vi "Ecrire_fichier_rapport_profil_EPC3000.vi"(1 "Commentaires":string, 4 "Chemin du fichier rapport":path) -> (5 "annulé":bool, 7 "error out":errorcluster caption="sortie d'erreur")   [LabVIEW 2022 SP3]
uses:
  Enum/Enum r3.ctl
  <vilib>/Utility/miscctls.llb/LVDateTimeRec.ctl
  <vilib>/printing/EasyPrintingControls.llb/layout_options.ctl
  <vilib>/printing/EasyPrintingControls.llb/orientation.ctl
  <vilib>/printing/EasyPrintingControls.llb/panel_scaling_for_page.ctl
  <vilib>/printing/EasyPrintingControls.llb/margins.ctl
  <vilib>/printing/EasyPrintingControls.llb/margin_values.ctl
  <vilib>/printing/EasyPrintingControls.llb/measurement_system.ctl
  <vilib>/printing/EasyPrintingControls.llb/printer_options.ctl
  <vilib>/printing/EasyPrintingControls.llb/printing_method.ctl
  <vilib>/printing/EasyPrintingControls.llb/color_or_monochrome.ctl
  <vilib>/printing/EasyPrintingControls.llb/page_header_options.ctl
  <vilib>/printing/EasyPrintingControls.llb/page_headers.ctl
  <vilib>/printing/EasyPrintingControls.llb/page_header_content_options.ctl
  <vilib>/printing/EasyPrintingControls.llb/contents.ctl
  <vilib>/printing/EasyPrintingControls.llb/report_type.ctl
  <vilib>/Utility/NIReport.llb/HTML Report Image Alignment.ctl
  Variables globales/Variables glob EUROTHERM.vi
  <vilib>/printing/EasyPrinting.llb/Print VI Panel or Documentation (path).vi
  <vilib>/Utility/NIReport.llb/Append Report Text (str wrap).vi
  <vilib>/Utility/NIReport.llb/Append Image to Report (path wrap).vi
  <vilib>/Utility/NIReport.llb/NI_report.lvclass
  <vilib>/Utility/NIReport.llb/NI_ReportGenerationCore.lvlib
panel:
  in  "Annuler lecture reg":bool
  in  "imprimer":bool
  in  "Bascule":bool
  out "nb profils":i32
  in  "Commande onglets":T1(tab)
  in  "Tinit reg 1":u16(ring) caption="Tinit sur reg :" items=["centre", "arrière"]
  out "Graph 1":cluster{"Y":dbl[], "Y":dbl[]}[](graph) caption="Profil"
  out "Régulateurs 1":string[](array[string]) caption="Régulateurs"
  out "Listing - 1":string caption="Listing programmes"
  out "Graph 2":cluster{"Y":dbl[], "Y":dbl[]}[](graph) caption="Profil"
  out "Régulateurs 2":string[](array[string]) caption="Régulateurs"
  in  "Tinit reg 2":u16(ring) caption="Tinit sur reg :" items=["EPC3008"]
  out "Listing - 2":string caption="Listing programmes"
  in  "Tinit reg 3":u16(ring) caption="Tinit sur reg :"
  out "Graph 3":cluster{"Y":dbl[], "Y":dbl[]}[](graph) caption="Profil"
  out "Régulateurs 3":string[](array[string]) caption="Régulateurs"
  out "Listing - 3":string caption="Listing programmes"
  in  "Tinit reg 4":u16(ring) caption="Tinit sur reg :"
  out "Graph 4":cluster{"Y":dbl[], "Y":dbl[]}[](graph) caption="Profil"
  out "Régulateurs 4":string[](array[string]) caption="Régulateurs"
  out "Listing - 4":string caption="Listing programmes"
  in  "Tinit reg 5":u16(ring) caption="Tinit sur reg :"
  out "Graph 5":cluster{"Y":dbl[], "Y":dbl[]}[](graph) caption="Profil"
  out "Régulateurs 5":string[](array[string]) caption="Régulateurs"
  out "Listing - 5":string caption="Listing programmes"
  in  "Tinit reg 6":u16(ring) caption="Tinit sur reg :"
  out "Graph 6":cluster{"Y":dbl[], "Y":dbl[]}[](graph) caption="Profil"
  out "Régulateurs 6":string[](array[string]) caption="Régulateurs"
  out "Listing - 6":string caption="Listing programmes"
  in  "Tinit reg 7":u16(ring) caption="Tinit sur reg :"
  out "Graph 7":cluster{"Y":dbl[], "Y":dbl[]}[](graph) caption="Profil"
  out "Régulateurs 7":string[](array[string]) caption="Régulateurs"
  out "Listing - 7":string caption="Listing programmes"
  in  "Tinit reg 8":u16(ring) caption="Tinit sur reg :"
  out "Graph 8":cluster{"Y":dbl[], "Y":dbl[]}[](graph) caption="Profil"
  out "Régulateurs 8":string[](array[string]) caption="Régulateurs"
  out "Listing - 8":string caption="Listing programmes"
  in  "Tinit reg 9":u16(ring) caption="Tinit sur reg :"
  out "Graph 9":cluster{"Y":dbl[], "Y":dbl[]}[](graph) caption="Profil"
  out "Régulateurs 9":string[](array[string]) caption="Régulateurs"
  out "Listing - 9":string caption="Listing programmes"
  in  "Tinit reg 10":u16(ring) caption="Tinit sur reg :"
  out "Graph 10":cluster{"Y":dbl[], "Y":dbl[]}[](graph) caption="Profil"
  out "Régulateurs 10":string[](array[string]) caption="Régulateurs"
  out "Listing - 10":string caption="Listing programmes"
  out "fichiers images":path[](array[path])
  in  "Annuler":bool
  in  "OK":bool
  out "Listings":string[](array[string])
  out "Profils":T2(array[cluster])
  out "Chaîne":string
  # "Ce logiciel et les informations qu'il contient, sont la propriété de l’IAS et ne peuvent être diffusés sans l’autorisation de la Station d’étalonnage"
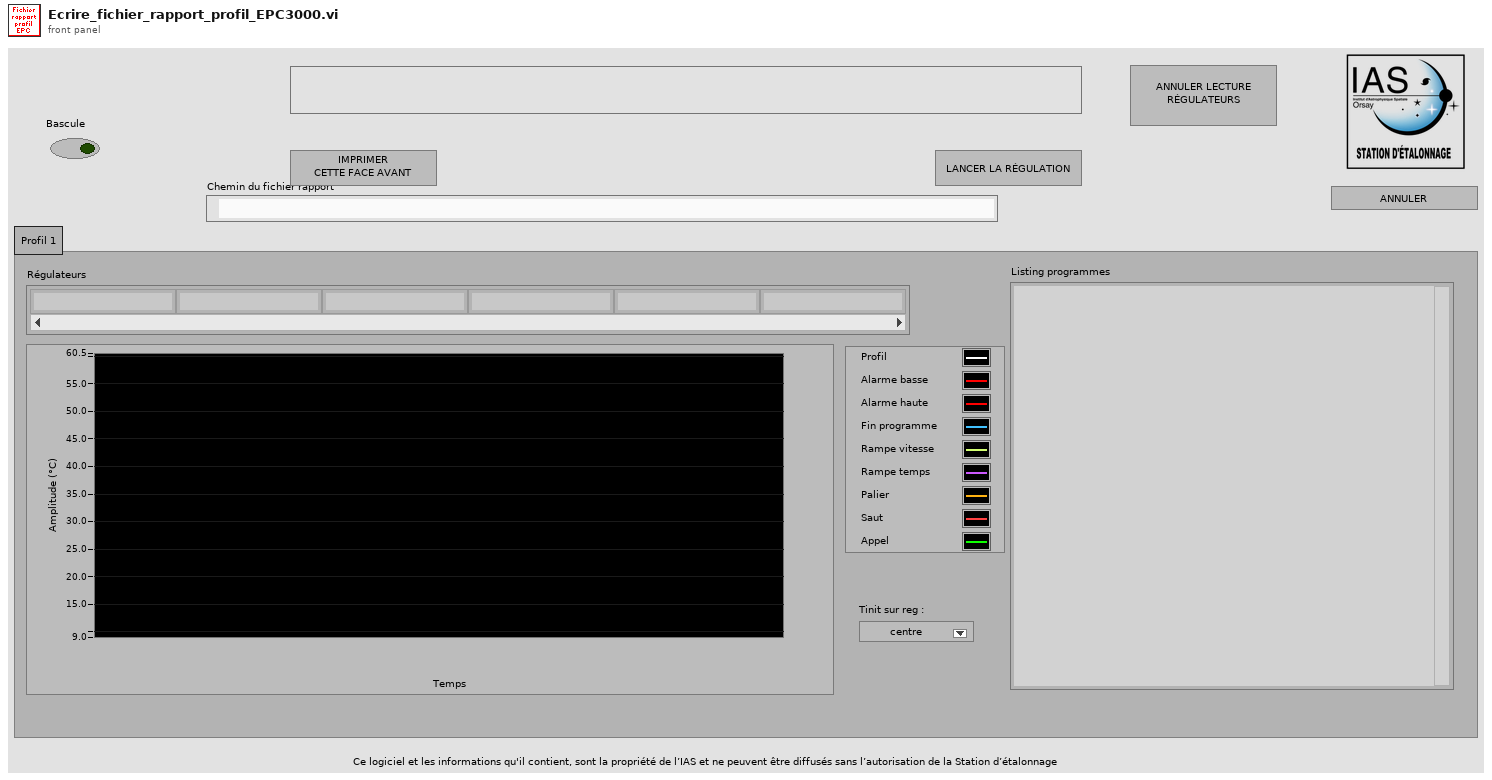
[diagram p1: front panel]
types:
  T1 = enum32{"Profil 1", "Profil 2", "Profil 3", "Profil 4", "Profil 5", "Profil 6", "Profil 7", "Profil 8", "Profil 9", "Profil 10"}
  T2 = cluster{"Config + Programmes":cluster{"Programmation configuration":cluster{"Command (PV)":string, dbl}[], "Programme 1":cluster{"chaîne o":string, "Received Value":dbl}[][], "Programme 2":cluster{"chaîne o":string, "Received Value":dbl}[][], "Programme 3":cluster{"chaîne o":string, "Received Value":dbl}[][], "Programme 4":cluster{"chaîne o":string, "Received Value":dbl}[][], "Programme 5":cluster{"chaîne o":string, "Received Value":dbl}[][], "Programme 6":cluster{"chaîne o":string, "Received Value":dbl}[][], "Programme 7":cluster{"chaîne o":string, "Received Value":dbl}[][], "Programme 8":cluster{"chaîne o":string, "Received Value":dbl}[][], "Programme 9":cluster{"chaîne o":string, "Received Value":dbl}[][], "Programme 10":cluster{"chaîne o":string, "Received Value":dbl}[][]}, "Régulateur":cluster{"Nom":string, "COM":refnum<visa-resource-name>, "Adresse":u8}[]}[]
  T3 = typedef "Enum r3.ctl" = enum16{"init", "différents profils", "graphs et listings", "validation", "fichiers images graph", "fichier html", "fin"}
  T4 = typedef "LVDateTimeRec.ctl" = cluster{"fractional second":dbl, "second":i32, "minute":i32, "hour":i32, "day of month":i32, "month":i32, "year":i32, "day of week":i32, "day of year":i32, "DST":i32}
  T5 = typedef "NI_ReportGenerationCore.lvlib/layout_options.ctl" = cluster{"orientation (unchanged)":T6, "panel scaling for page (unchanged)":T7, "margins":T8, "printer options":T11, "page header options":T14}
  T6 = typedef "NI_ReportGenerationCore.lvlib/orientation.ctl" = u16
  T7 = typedef "NI_ReportGenerationCore.lvlib/panel_scaling_for_page.ctl" = u16
  T8 = typedef "NI_ReportGenerationCore.lvlib/margins.ctl" = cluster{"override VI margins (false)":bool, "margins (1.00)":T9, "measurement system (default)":T10}
  T9 = typedef "NI_ReportGenerationCore.lvlib/margin_values.ctl" = cluster{"top":dbl, "left":dbl, "right":dbl, "bottom":dbl}
  T10 = typedef "NI_ReportGenerationCore.lvlib/measurement_system.ctl" = u16
  T11 = typedef "NI_ReportGenerationCore.lvlib/printer_options.ctl" = cluster{"destination printer name (current)":string, "printing method (unchanged)":T12, "color or monochrome (unchanged)":T13}
  T12 = typedef "NI_ReportGenerationCore.lvlib/printing_method.ctl" = u16
  T13 = typedef "NI_ReportGenerationCore.lvlib/color_or_monochrome.ctl" = u16
  T14 = typedef "NI_ReportGenerationCore.lvlib/page_header_options.ctl" = cluster{"page headers (unchanged)":T15, "page header content options":T16}
  T15 = typedef "NI_ReportGenerationCore.lvlib/page_headers.ctl" = u16
  T16 = typedef "NI_ReportGenerationCore.lvlib/page_header_content_options.ctl" = cluster{"Include VI Name":bool, "Include VI Path":bool, "Include Last Modification Date":bool, "Include Date Printed":bool, "Include Page Number":bool, "Include VI Icon":bool}
  T17 = enum16{"Standard Report", "HTML", "Word", "Excel"}
  T18 = typedef "NI_ReportGenerationCore.lvlib/HTML Report Image Alignment.ctl" = enum16{"(default)", "LEFT", "RIGHT", "TOP", "TEXTTOP", "MIDDLE", "ABSMIDDLE", "BASELINE", "BOTTOM", "ABSBOTTOM"}
  T19 = cluster{"Programmation configuration":cluster{"Command (PV)":string, dbl}[], "Programme 1":cluster{"chaîne o":string, "Received Value":dbl}[][], "Programme 2":cluster{"chaîne o":string, "Received Value":dbl}[][], "Programme 3":cluster{"chaîne o":string, "Received Value":dbl}[][], "Programme 4":cluster{"chaîne o":string, "Received Value":dbl}[][], "Programme 5":cluster{"chaîne o":string, "Received Value":dbl}[][], "Programme 6":cluster{"chaîne o":string, "Received Value":dbl}[][], "Programme 7":cluster{"chaîne o":string, "Received Value":dbl}[][], "Programme 8":cluster{"chaîne o":string, "Received Value":dbl}[][], "Programme 9":cluster{"chaîne o":string, "Received Value":dbl}[][], "Programme 10":cluster{"chaîne o":string, "Received Value":dbl}[][]}
  T20 = cluster{cluster{"Programmation configuration":cluster{"Command (PV)":string, dbl}[], "Programme 1":cluster{"chaîne o":string, "Received Value":dbl}[][], "Programme 2":cluster{"chaîne o":string, "Received Value":dbl}[][], "Programme 3":cluster{"chaîne o":string, "Received Value":dbl}[][], "Programme 4":cluster{"chaîne o":string, "Received Value":dbl}[][], "Programme 5":cluster{"chaîne o":string, "Received Value":dbl}[][], "Programme 6":cluster{"chaîne o":string, "Received Value":dbl}[][], "Programme 7":cluster{"chaîne o":string, "Received Value":dbl}[][], "Programme 8":cluster{"chaîne o":string, "Received Value":dbl}[][], "Programme 9":cluster{"chaîne o":string, "Received Value":dbl}[][], "Programme 10":cluster{"chaîne o":string, "Received Value":dbl}[][]}[]}
  T21 = cluster{"Nom":string, "COM":refnum<visa-resource-name>, "Adresse":u8}[]
  T22 = cluster{"Nom":string, "COM":refnum<visa-resource-name>, "Adresse":u8}
  T23 = cluster{"Ev_Saut":dbl[], "Ev_Palier":dbl[], "Ev_Rampe_vitesse":dbl[], "Ev_Rampe_temps":dbl[], "Ev_Appel":dbl[], "Ev_Fin":dbl[], "T_Fin":dbl[], "T_Appel":dbl[], "T_Rampe_temps":dbl[], "T_Rampe_vitesse":dbl[], "T_Palier":dbl[], "T_Saut":dbl[], "Type de fin":string}
  T24 = cluster{"chaîne o":string, "Received Value":dbl}[][]
  T25 = cluster{"Tempé. max":dbl, "Tempé. min":dbl, "Temps max":dbl, "Temps min":dbl}
  T26 = cluster{"Config + Programmes":cluster{"Programmation configuration":cluster{"Command (PV)":string, dbl}[], "Programme 1":cluster{"chaîne o":string, "Received Value":dbl}[][], "Programme 2":cluster{"chaîne o":string, "Received Value":dbl}[][], "Programme 3":cluster{"chaîne o":string, "Received Value":dbl}[][], "Programme 4":cluster{"chaîne o":string, "Received Value":dbl}[][], "Programme 5":cluster{"chaîne o":string, "Received Value":dbl}[][], "Programme 6":cluster{"chaîne o":string, "Received Value":dbl}[][], "Programme 7":cluster{"chaîne o":string, "Received Value":dbl}[][], "Programme 8":cluster{"chaîne o":string, "Received Value":dbl}[][], "Programme 9":cluster{"chaîne o":string, "Received Value":dbl}[][], "Programme 10":cluster{"chaîne o":string, "Received Value":dbl}[][]}, "Régulateur":cluster{"Nom":string, "COM":refnum<visa-resource-name>, "Adresse":u8}[]}
  T27 = typedef "NI_ReportGenerationCore.lvlib/report_type.ctl" = u16
  T28 = typedef "NI_ReportGenerationCore.lvlib/contents.ctl" = u16
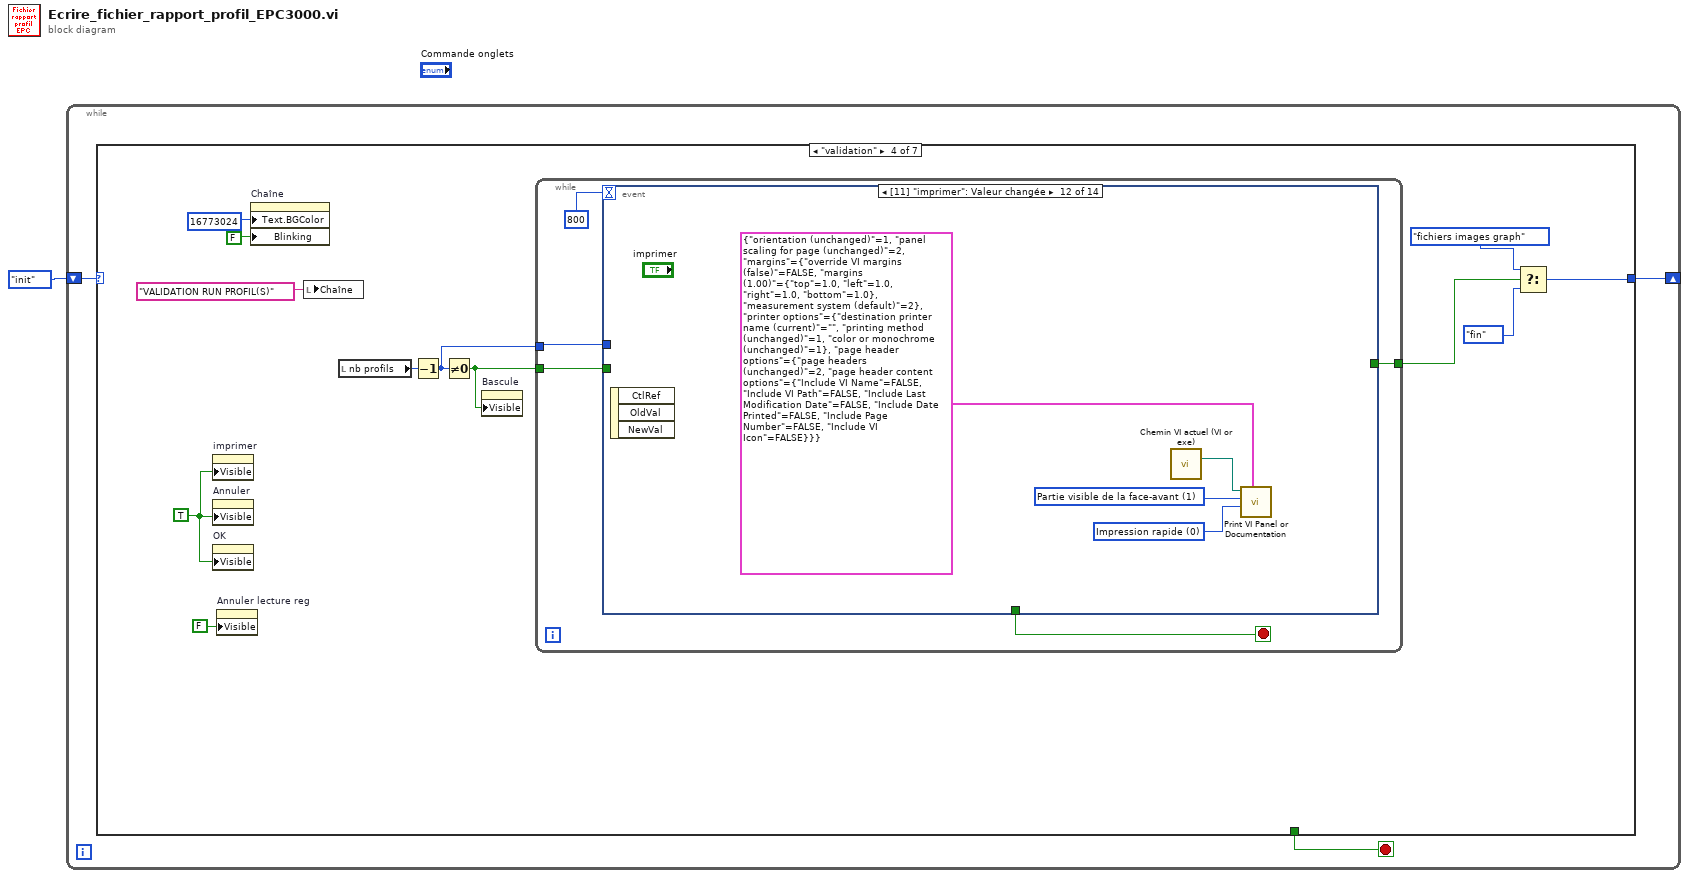
[diagram p0: block diagram]
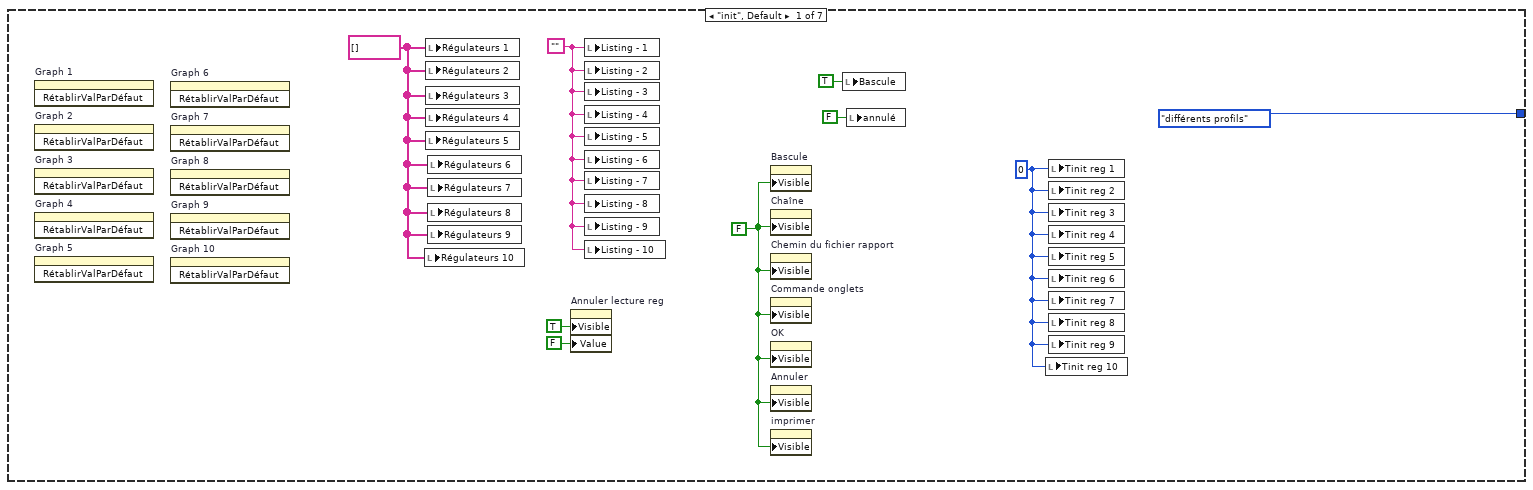
[diagram p2: hidden frame]
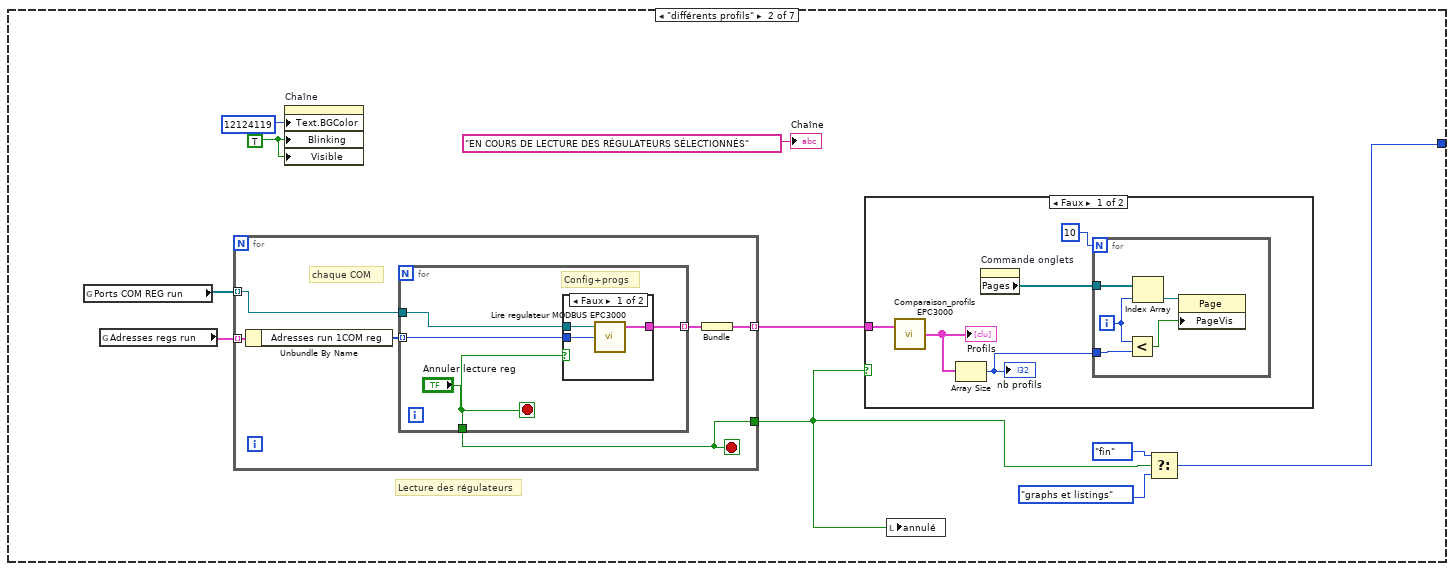
[diagram p3: hidden frame]
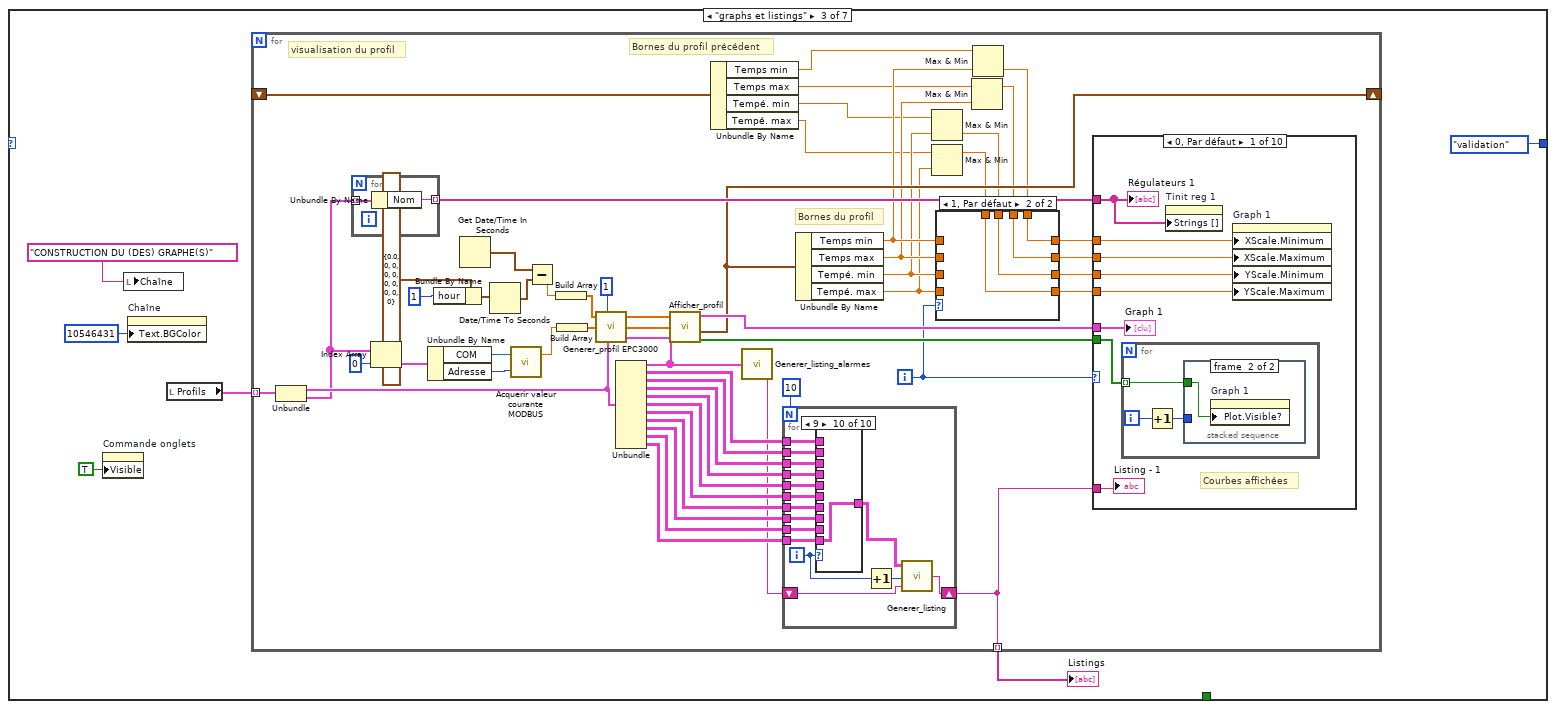
[diagram p6: hidden frame]
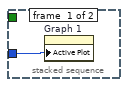
[diagram p17: hidden frame]
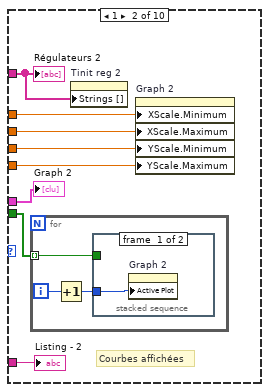
[diagram p18: hidden frame]
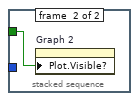
[diagram p19: hidden frame]
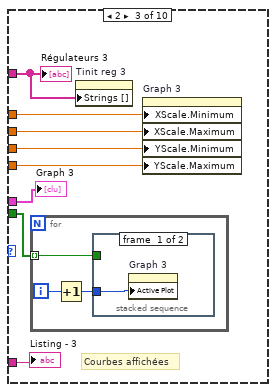
[diagram p20: hidden frame]
diagram:
  n1 = while {
    shift-right: [w3] -> _
    shift-left: Enum_r3."init" ("Énum") -> [w4]
    stop <- w2 stop-if-true
    n2 = case shown="\"validation\"" w4 {
      tunnel: [Enum_r3."différents profils" ("Énum") w15 Enum_r3."validation" ("Énum") w283 Enum_r3."fichier html" ("Énum") Enum_r3."fin" ("Énum") Enum_r3."init" ("Énum")] -> w3
      tunnel: [_ _ _ _ _ _ TRUE] -> w2
      frame "init", Default {
        w8 = ""
        w9 = u16 0
        w11 = string[] [] ("Régulateurs 1")
        w7 = FALSE ("Visible")
        n3 = invoke on="Graph 1" class="GraphXY (strict)" method="RétablirValParDéfaut"() -> ()  [unwired: 3 in, 3 out]
        n4 = invoke on="Graph 2" class="GraphXY (strict)" method="RétablirValParDéfaut"() -> ()  [unwired: 3 in, 3 out]
        n5 = invoke on="Graph 3" class="GraphXY (strict)" method="RétablirValParDéfaut"() -> ()  [unwired: 3 in, 3 out]
        n6 = invoke on="Graph 4" class="GraphXY (strict)" method="RétablirValParDéfaut"() -> ()  [unwired: 3 in, 3 out]
        n7 = invoke on="Graph 5" class="GraphXY (strict)" method="RétablirValParDéfaut"() -> ()  [unwired: 3 in, 3 out]
        n8 = invoke on="Graph 6" class="GraphXY (strict)" method="RétablirValParDéfaut"() -> ()  [unwired: 3 in, 3 out]
        n9 = invoke on="Graph 7" class="GraphXY (strict)" method="RétablirValParDéfaut"() -> ()  [unwired: 3 in, 3 out]
        n10 = invoke on="Graph 8" class="GraphXY (strict)" method="RétablirValParDéfaut"() -> ()  [unwired: 3 in, 3 out]
        n11 = invoke on="Graph 9" class="GraphXY (strict)" method="RétablirValParDéfaut"() -> ()  [unwired: 3 in, 3 out]
        n12 = invoke on="Graph 10" class="GraphXY (strict)" method="RétablirValParDéfaut"() -> ()  [unwired: 3 in, 3 out]
        n13 = local write "Régulateurs 10"(w11) -> ()
        n14 = local write "Régulateurs 1"(w11) -> ()
        n15 = local write "Régulateurs 2"(w11) -> ()
        n16 = local write "Régulateurs 3"(w11) -> ()
        n17 = local write "Régulateurs 4"(w11) -> ()
        n18 = local write "Régulateurs 5"(w11) -> ()
        n19 = local write "Régulateurs 6"(w11) -> ()
        n20 = local write "Régulateurs 7"(w11) -> ()
        n21 = local write "Régulateurs 8"(w11) -> ()
        n22 = local write "Régulateurs 9"(w11) -> ()
        n23 = property on="Annuler lecture reg" class="Bool (strict)"("Visible"=TRUE, "Value"=FALSE ("Annuler lecture reg")) -> ()  [unwired: 2 in, 2 out]
        n24 = local write "Listing - 1"(w8) -> ()
        n25 = local write "Listing - 2"(w8) -> ()
        n26 = local write "Listing - 3"(w8) -> ()
        n27 = local write "Listing - 4"(w8) -> ()
        n28 = local write "Listing - 5"(w8) -> ()
        n29 = local write "Listing - 6"(w8) -> ()
        n30 = local write "Listing - 7"(w8) -> ()
        n31 = local write "Listing - 8"(w8) -> ()
        n32 = local write "Listing - 9"(w8) -> ()
        n33 = local write "Listing - 10"(w8) -> ()
        n34 = property on="Bascule" class="Bool (strict)"("Visible"=w7) -> ()  [unwired: 2 in, 2 out]
        n35 = property on="Chaîne" class="Ch"("Visible"=w7) -> ()  [unwired: 2 in, 2 out]
        n36 = property on="Chemin du fichier rapport" class="Chm"("Visible"=w7) -> ()  [unwired: 2 in, 2 out]
        n37 = property on="Commande onglets" class="Onglet (strict)"("Visible"=w7) -> ()  [unwired: 2 in, 2 out]
        n38 = property on="OK" class="Bool"("Visible"=w7) -> ()  [unwired: 2 in, 2 out]
        n39 = property on="Annuler" class="Bool"("Visible"=w7) -> ()  [unwired: 2 in, 2 out]
        n40 = property on="imprimer" class="Bool"("Visible"=w7) -> ()  [unwired: 2 in, 2 out]
        n41 = local write "Bascule"(TRUE ("Bascule")) -> ()
        n42 = local write "annulé"(FALSE ("annulé")) -> ()
        n43 = local write "Tinit reg 10"(w9) -> ()
        n44 = local write "Tinit reg 1"(w9) -> ()
        n45 = local write "Tinit reg 2"(w9) -> ()
        n46 = local write "Tinit reg 3"(w9) -> ()
        n47 = local write "Tinit reg 4"(w9) -> ()
        n48 = local write "Tinit reg 5"(w9) -> ()
        n49 = local write "Tinit reg 6"(w9) -> ()
        n50 = local write "Tinit reg 7"(w9) -> ()
        n51 = local write "Tinit reg 8"(w9) -> ()
        n52 = local write "Tinit reg 9"(w9) -> ()
      }
      frame "différents profils" {
        w19 = TRUE ("Clignotant")
        # "Lecture des régulateurs"
        n53 = global read "Variables glob EUROTHERM.vi" "Ports COM REG run"() -> (w18:refnum<visa-resource-name>[])
        n54 = global read "Variables glob EUROTHERM.vi" "Adresses regs run"() -> (w22:cluster{"Adresses run 1COM reg":u16[]}[])
        n55 = for {
          tunnel: [w38] -> w23 mode=indexing
          tunnel: w22 -> [w37] mode=indexing
          tunnel: w18 -> [w35] mode=indexing
          tunnel: [w34] -> w14
          stop <- w34 stop-if-true
          # "chaque COM"
          n56 = Unbundle By Name(w37) -> ("Adresses run 1COM reg"=w36:u16[])
          n57 = for {
            tunnel: w36 -> [w42] mode=indexing
            tunnel: [w41] -> w39 mode=indexing
            tunnel: w35 -> [w43]
            tunnel: ["Annuler lecture reg"] -> w34
            stop <- "Annuler lecture reg" stop-if-true
            # "Config+progs"
            n58 = case shown="Faux" "Annuler lecture reg" {
              tunnel: w43 -> [w46 _]
              tunnel: w42 -> [w45 _]
              tunnel: [w44 _] -> w41
              frame False {
                n59 = call "Lire regulateur MODBUS EPC3000.vi"("Adresse régulateur"=w45, "Port COM run 1 REG"=w46) -> ("Config + Programmes"=w44:T19)  [unwired: 2 in, 1 out]
              }
              frame True {
              }
            }
          }
          n60 = Bundle(w39) -> (w38:T20)  [unwired: 1 in]
        }
        n61 = property on="Chaîne" class="Ch"("Text.BGColor"=u32 12124119 ("Texte.Couleurs du texte:Arrière-plan"), "Blinking"=w19, "Visible"=w19) -> ()  [unwired: 2 in, 2 out]
        n62 = case shown="Faux" w14 {
          tunnel: w23 -> [w28 _]
          frame False {
            n63 = call "Comparaison_profils EPC3000.vi"("Configs + progs régulateurs"=w28) -> ("Profils"=w27:T2)  [unwired: 2 in]
            "Profils" <- w27
            n64 = Array Size(array=w27) -> (size(s)=w25:i32)
            "nb profils" <- w25
            n65 = property on="Commande onglets" class="Onglet (strict)"() -> ("Pages"=w26:refnum<vi>[])  [unwired: 2 in, 2 out]
            n66 = for {
              N: 10 -> [_]
              tunnel: w26 -> [w33]
              tunnel: w25 -> [w30]
              i -> [w31]
              n67 = Less?(x=w31, y=w30) -> (x < y?=w29:bool)
              n68 = Index Array(array=w33, index=w31) -> (element=w32:refnum<vi>)
              n69 = property class="Page"(reference=w32, "PageVis"=w29) -> ()  [unwired: 1 in, 2 out]
            }
          }
          frame True {
          }
        }
        n70 = local write "annulé"(w14) -> ()
        n71 = Select(t=Enum_r3."fin" ("Énum"), s=w14, f=Enum_r3."graphs et listings" ("Énum")) -> (s? t:f=w15:T3)
        "Chaîne" <- "EN COURS DE LECTURE DES RÉGULATEURS SÉLECTIONNÉS" ("Chaîne")
      }
      frame "graphs et listings" {
        n72 = property on="Commande onglets" class="Onglet (strict)"("Visible"=TRUE) -> ()  [unwired: 2 in, 2 out]
        n73 = local write "Chaîne"("CONSTRUCTION DU (DES) GRAPHE(S)" ("Chaîne")) -> ()
        n74 = property on="Chaîne" class="Ch"("Text.BGColor"=u32 10546431 ("Texte.Couleurs du texte:Arrière-plan")) -> ()  [unwired: 2 in, 2 out]
        n75 = local read "Profils"() -> (w52:T2)
        n76 = for {
          tunnel: w52 -> [w89] mode=indexing
          tunnel: [w74] -> w51 mode=indexing
          shift-right: [w71] -> _
          shift-left: _ -> [w70]
          i -> [w63]
          # "Bornes du profil précédent"
          # "Bornes du profil"
          # "visualisation du profil"
          n77 = Unbundle(w89) -> ("Config + Programmes"=w104:T19, "Régulateur"=w88:T21)
          n78 = for {
            tunnel: w88 -> [w273] mode=indexing
            tunnel: [w272] -> w85 mode=indexing
            n79 = Unbundle By Name(w273) -> ("Nom"=w272:string)
          }
          n80 = Index Array(array=w88, index=0 ("indice")) -> (element=w106:T22)
          n81 = Unbundle By Name(w106) -> ("COM"=w107:refnum<visa-resource-name>, "Adresse"=w108:u8)
          n82 = Bundle By Name(cluster=T4 {"fractional second"=0.0, "second"=0, "minute"=0, "hour"=0, "day of month"=0, "month"=0, "year"=0, "day of week"=0, "day of year"=0, "DST"=0} ("cluster date/heure"), "hour"=1) -> (w98:T4)
          n83 = Get Date/Time In Seconds() -> (seconds since 1Jan1904=w90:timestamp)
          n84 = Date/Time To Seconds(2:w98) -> (0:w95:timestamp)  [unwired: 1 in]
          n85 = call "Acquerir valeur courante MODBUS.vi"("Adresse régulateur"=w108, "Port COM run 1 REG"=w107) -> ("Température"=w102:dbl)  [unwired: 1 out]
          n86 = Subtract(x=w90, y=w95) -> (x-y=w97:dbl)
          n87 = Build Array(w97) -> (w100:dbl[])
          n88 = Build Array(w102) -> (w101:dbl[])
          n89 = call "Generer_profil EPC3000.vi"("Temps (s)"=w100, "Num_Prog"=u8 1, "Températures (°C)"=w101, "Programmes et config"=w104) -> ("Temps (s)"=w93:dbl[], "Températures (°C)"=w92:dbl[], "Evennements_sortie"=w91:T23)  [unwired: 1 in]
          n90 = Unbundle(w104) -> ("Programmation configuration"=w103:cluster{"Command (PV)":string, dbl}[], "Programme 1"=w75:T24, "Programme 2"=w76:T24, "Programme 3"=w77:T24, "Programme 4"=w78:T24, "Programme 5"=w79:T24, "Programme 6"=w80:T24, "Programme 7"=w81:T24, "Programme 8"=w82:T24, "Programme 9"=w83:T24, "Programme 10"=w84:T24)
          n91 = call "Afficher_profil.vi"("Configuration"=w103, "Temps (s)"=w93, "Températures (°C)"=w92, "Evennements_entrée"=w91) -> ("Graphe XY"=w86:cluster{"Y":dbl[], "Y":dbl[]}[], "Bornes profil"=w71:T25, "Courbes à afficher"=w87:bool[])  [unwired: 1 out]
          n92 = Unbundle By Name(w70) -> ("Temps min"=w69:dbl, "Temps max"=w61:dbl, "Tempé. min"=w58:dbl, "Tempé. max"=w55:dbl)
          n93 = call "Generer_listing_alarmes.vi"("Configuration"=w103) -> ("Listing alarmes"=w73:string)
          n94 = for {
            N: 10 -> [_]
            tunnel: w84 -> [w122]
            tunnel: w83 -> [w123]
            tunnel: w82 -> [w124]
            tunnel: w81 -> [w125]
            tunnel: w80 -> [w126]
            tunnel: w79 -> [w127]
            tunnel: w78 -> [w128]
            tunnel: w77 -> [w129]
            tunnel: w76 -> [w130]
            tunnel: w75 -> [w131]
            shift-right: [w118] -> w74
            shift-left: w73 -> [w117]
            i -> [w119]
            n95 = case shown="9" w119 {
              tunnel: w131 -> [w132 _ _ _ _ _ _ _ _ _]
              tunnel: w130 -> [_ w133 _ _ _ _ _ _ _ _]
              tunnel: w129 -> [_ _ w134 _ _ _ _ _ _ _]
              tunnel: w128 -> [_ _ _ w135 _ _ _ _ _ _]
              tunnel: w127 -> [_ _ _ _ w136 _ _ _ _ _]
              tunnel: w126 -> [_ _ _ _ _ w137 _ _ _ _]
              tunnel: w125 -> [_ _ _ _ _ _ w138 _ _ _]
              tunnel: w124 -> [_ _ _ _ _ _ _ w139 _ _]
              tunnel: w123 -> [_ _ _ _ _ _ _ _ w140 _]
              tunnel: w122 -> [_ _ _ _ _ _ _ _ _ w141]
              tunnel: [w132 w133 w134 w135 w136 w137 w138 w139 w140 w141] -> w121
              frame 0, Default {
              }
              frame 1 {
              }
              frame 2 {
              }
              frame 3 {
              }
              frame 4 {
              }
              frame 5 {
              }
              frame 6 {
              }
              frame 7 {
              }
              frame 8 {
              }
              frame 9 {
              }
            }
            n96 = Increment(x=w119) -> (x+1=w120:i32)
            n97 = call "Generer_listing.vi"("Listing_entrée"=w117, "Numéro de programme"=w120, "Programme"=w121) -> ("Listing_sortie"=w118:string)
          }
          n98 = Unbundle By Name(w71) -> ("Temps min"=w68:dbl, "Temps max"=w60:dbl, "Tempé. min"=w57:dbl, "Tempé. max"=w54:dbl)
          n99 = Max & Min(x=w58, y=w57) -> (min(x,y)=w56:dbl)  [unwired: 1 out]
          n100 = Max & Min(x=w55, y=w54) -> (max(x,y)=w53:dbl)  [unwired: 1 out]
          n101 = Max & Min(x=w61, y=w60) -> (max(x,y)=w59:dbl)  [unwired: 1 out]
          n102 = Max & Min(x=w69, y=w68) -> (min(x,y)=w62:dbl)  [unwired: 1 out]
          n103 = case shown="1, Par défaut" w63 {
            tunnel: w68 -> [w112 _]
            tunnel: [w112 w116] -> w67
            tunnel: w60 -> [w111 _]
            tunnel: [w111 w115] -> w66
            tunnel: w57 -> [w110 _]
            tunnel: [w110 w114] -> w65
            tunnel: w54 -> [w109 _]
            tunnel: [w109 w113] -> w64
            tunnel: w62 -> [_ w116]
            tunnel: w59 -> [_ w115]
            tunnel: w56 -> [_ w114]
            tunnel: w53 -> [_ w113]
            frame 0 {
            }
            frame 1, Default {
            }
          }
          n104 = case shown="0, Par défaut" w63 {
            tunnel: w87 -> [w149 w161 w174 w187 w200 w214 w227 w240 w253 w266]
            tunnel: w85 -> [w147 w160 w173 w186 w199 w212 w225 w238 w251 w264]
            tunnel: w86 -> [w148 w162 w175 w188 w201 w213 w226 w239 w252 w265]
            tunnel: w74 -> [w146 w159 w172 w185 w198 w211 w224 w237 w250 w263]
            tunnel: w67 -> [w145 w158 w171 w184 w197 w210 w223 w236 w249 w262]
            tunnel: w66 -> [w144 w157 w170 w183 w196 w209 w222 w235 w248 w261]
            tunnel: w65 -> [w143 w156 w169 w182 w195 w208 w221 w234 w247 w260]
            tunnel: w64 -> [w142 w155 w168 w181 w194 w207 w220 w233 w246 w259]
            frame 0, Default {
              # "Courbes affichées"
              n105 = for {
                tunnel: w149 -> [w150] mode=indexing
                i -> [w151]
                n106 = Increment(x=w151) -> (x+1=w152:i32)
                n107 = stacked-sequence {
                  tunnel: w150 -> [_ w154]
                  tunnel: w152 -> [w153 _]
                  frame #0 {
                    n108 = property on="Graph 1" class="GraphXY (strict)"("Active Plot"=w153) -> ()  [unwired: 2 in, 2 out]
                  }
                  frame #1 {
                    n109 = property on="Graph 1" class="GraphXY (strict)"("Plot.Visible?"=w154) -> ()  [unwired: 2 in, 2 out]
                  }
                }
              }
              n110 = property on="Tinit reg 1" class="MDér (strict)"("Strings []"=w147) -> ()  [unwired: 2 in, 2 out]
              n111 = property on="Graph 1" class="GraphXY (strict)"("XScale.Minimum"=w145, "XScale.Maximum"=w144, "YScale.Minimum"=w143, "YScale.Maximum"=w142) -> ()  [unwired: 2 in, 2 out]
              "Régulateurs 1" <- w147
              "Graph 1" <- w148
              "Listing - 1" <- w146
            }
            frame 1 {
              # "Courbes affichées"
              n112 = for {
                tunnel: w161 -> [w163] mode=indexing
                i -> [w164]
                n113 = Increment(x=w164) -> (x+1=w165:i32)
                n114 = stacked-sequence {
                  tunnel: w163 -> [_ w167]
                  tunnel: w165 -> [w166 _]
                  frame #0 {
                    n115 = property on="Graph 2" class="GraphXY (strict)"("Active Plot"=w166) -> ()  [unwired: 2 in, 2 out]
                  }
                  frame #1 {
                    n116 = property on="Graph 2" class="GraphXY (strict)"("Plot.Visible?"=w167) -> ()  [unwired: 2 in, 2 out]
                  }
                }
              }
              n117 = property on="Tinit reg 2" class="MDér (strict)"("Strings []"=w160) -> ()  [unwired: 2 in, 2 out]
              n118 = property on="Graph 2" class="GraphXY (strict)"("XScale.Minimum"=w158, "XScale.Maximum"=w157, "YScale.Minimum"=w156, "YScale.Maximum"=w155) -> ()  [unwired: 2 in, 2 out]
              "Régulateurs 2" <- w160
              "Graph 2" <- w162
              "Listing - 2" <- w159
            }
            frame 2 {
              # "Courbes affichées"
              n119 = for {
                tunnel: w174 -> [w176] mode=indexing
                i -> [w177]
                n120 = Increment(x=w177) -> (x+1=w178:i32)
                n121 = stacked-sequence {
                  tunnel: w176 -> [_ w180]
                  tunnel: w178 -> [w179 _]
                  frame #0 {
                    n122 = property on="Graph 3" class="GraphXY (strict)"("Active Plot"=w179) -> ()  [unwired: 2 in, 2 out]
                  }
                  frame #1 {
                    n123 = property on="Graph 3" class="GraphXY (strict)"("Plot.Visible?"=w180) -> ()  [unwired: 2 in, 2 out]
                  }
                }
              }
              n124 = property on="Tinit reg 3" class="MDér (strict)"("Strings []"=w173) -> ()  [unwired: 2 in, 2 out]
              n125 = property on="Graph 3" class="GraphXY (strict)"("XScale.Minimum"=w171, "XScale.Maximum"=w170, "YScale.Minimum"=w169, "YScale.Maximum"=w168) -> ()  [unwired: 2 in, 2 out]
              "Régulateurs 3" <- w173
              "Graph 3" <- w175
              "Listing - 3" <- w172
            }
            frame 3 {
              # "Courbes affichées"
              n126 = for {
                tunnel: w187 -> [w189] mode=indexing
                i -> [w190]
                n127 = Increment(x=w190) -> (x+1=w191:i32)
                n128 = stacked-sequence {
                  tunnel: w189 -> [_ w193]
                  tunnel: w191 -> [w192 _]
                  frame #0 {
                    n129 = property on="Graph 4" class="GraphXY (strict)"("Active Plot"=w192) -> ()  [unwired: 2 in, 2 out]
                  }
                  frame #1 {
                    n130 = property on="Graph 4" class="GraphXY (strict)"("Plot.Visible?"=w193) -> ()  [unwired: 2 in, 2 out]
                  }
                }
              }
              n131 = property on="Tinit reg 4" class="MDér (strict)"("Strings []"=w186) -> ()  [unwired: 2 in, 2 out]
              n132 = property on="Graph 4" class="GraphXY (strict)"("XScale.Minimum"=w184, "XScale.Maximum"=w183, "YScale.Minimum"=w182, "YScale.Maximum"=w181) -> ()  [unwired: 2 in, 2 out]
              "Régulateurs 4" <- w186
              "Graph 4" <- w188
              "Listing - 4" <- w185
            }
            frame 4 {
              # "Courbes affichées"
              n133 = for {
                tunnel: w200 -> [w202] mode=indexing
                i -> [w203]
                n134 = Increment(x=w203) -> (x+1=w204:i32)
                n135 = stacked-sequence {
                  tunnel: w202 -> [_ w206]
                  tunnel: w204 -> [w205 _]
                  frame #0 {
                    n136 = property on="Graph 5" class="GraphXY (strict)"("Active Plot"=w205) -> ()  [unwired: 2 in, 2 out]
                  }
                  frame #1 {
                    n137 = property on="Graph 5" class="GraphXY (strict)"("Plot.Visible?"=w206) -> ()  [unwired: 2 in, 2 out]
                  }
                }
              }
              n138 = property on="Tinit reg 5" class="MDér (strict)"("Strings []"=w199) -> ()  [unwired: 2 in, 2 out]
              n139 = property on="Graph 5" class="GraphXY (strict)"("XScale.Minimum"=w197, "XScale.Maximum"=w196, "YScale.Minimum"=w195, "YScale.Maximum"=w194) -> ()  [unwired: 2 in, 2 out]
              "Régulateurs 5" <- w199
              "Graph 5" <- w201
              "Listing - 5" <- w198
            }
            frame 5 {
              # "Courbes affichées"
              n140 = for {
                tunnel: w214 -> [w215] mode=indexing
                i -> [w216]
                n141 = Increment(x=w216) -> (x+1=w217:i32)
                n142 = stacked-sequence {
                  tunnel: w215 -> [_ w219]
                  tunnel: w217 -> [w218 _]
                  frame #0 {
                    n143 = property on="Graph 6" class="GraphXY (strict)"("Active Plot"=w218) -> ()  [unwired: 2 in, 2 out]
                  }
                  frame #1 {
                    n144 = property on="Graph 6" class="GraphXY (strict)"("Plot.Visible?"=w219) -> ()  [unwired: 2 in, 2 out]
                  }
                }
              }
              n145 = property on="Tinit reg 6" class="MDér (strict)"("Strings []"=w212) -> ()  [unwired: 2 in, 2 out]
              n146 = property on="Graph 6" class="GraphXY (strict)"("XScale.Minimum"=w210, "XScale.Maximum"=w209, "YScale.Minimum"=w208, "YScale.Maximum"=w207) -> ()  [unwired: 2 in, 2 out]
              "Régulateurs 6" <- w212
              "Graph 6" <- w213
              "Listing - 6" <- w211
            }
            frame 6 {
              # "Courbes affichées"
              n147 = for {
                tunnel: w227 -> [w228] mode=indexing
                i -> [w229]
                n148 = Increment(x=w229) -> (x+1=w230:i32)
                n149 = stacked-sequence {
                  tunnel: w228 -> [_ w232]
                  tunnel: w230 -> [w231 _]
                  frame #0 {
                    n150 = property on="Graph 7" class="GraphXY (strict)"("Active Plot"=w231) -> ()  [unwired: 2 in, 2 out]
                  }
                  frame #1 {
                    n151 = property on="Graph 7" class="GraphXY (strict)"("Plot.Visible?"=w232) -> ()  [unwired: 2 in, 2 out]
                  }
                }
              }
              n152 = property on="Tinit reg 7" class="MDér (strict)"("Strings []"=w225) -> ()  [unwired: 2 in, 2 out]
              n153 = property on="Graph 7" class="GraphXY (strict)"("XScale.Minimum"=w223, "XScale.Maximum"=w222, "YScale.Minimum"=w221, "YScale.Maximum"=w220) -> ()  [unwired: 2 in, 2 out]
              "Régulateurs 7" <- w225
              "Graph 7" <- w226
              "Listing - 7" <- w224
            }
            frame 7 {
              # "Courbes affichées"
              n154 = for {
                tunnel: w240 -> [w241] mode=indexing
                i -> [w242]
                n155 = Increment(x=w242) -> (x+1=w243:i32)
                n156 = stacked-sequence {
                  tunnel: w241 -> [_ w245]
                  tunnel: w243 -> [w244 _]
                  frame #0 {
                    n157 = property on="Graph 8" class="GraphXY (strict)"("Active Plot"=w244) -> ()  [unwired: 2 in, 2 out]
                  }
                  frame #1 {
                    n158 = property on="Graph 8" class="GraphXY (strict)"("Plot.Visible?"=w245) -> ()  [unwired: 2 in, 2 out]
                  }
                }
              }
              n159 = property on="Tinit reg 8" class="MDér (strict)"("Strings []"=w238) -> ()  [unwired: 2 in, 2 out]
              n160 = property on="Graph 8" class="GraphXY (strict)"("XScale.Minimum"=w236, "XScale.Maximum"=w235, "YScale.Minimum"=w234, "YScale.Maximum"=w233) -> ()  [unwired: 2 in, 2 out]
              "Régulateurs 8" <- w238
              "Graph 8" <- w239
              "Listing - 8" <- w237
            }
            frame 8 {
              # "Courbes affichées"
              n161 = for {
                tunnel: w253 -> [w254] mode=indexing
                i -> [w255]
                n162 = Increment(x=w255) -> (x+1=w256:i32)
                n163 = stacked-sequence {
                  tunnel: w254 -> [_ w258]
                  tunnel: w256 -> [w257 _]
                  frame #0 {
                    n164 = property on="Graph 9" class="GraphXY (strict)"("Active Plot"=w257) -> ()  [unwired: 2 in, 2 out]
                  }
                  frame #1 {
                    n165 = property on="Graph 9" class="GraphXY (strict)"("Plot.Visible?"=w258) -> ()  [unwired: 2 in, 2 out]
                  }
                }
              }
              n166 = property on="Tinit reg 9" class="MDér (strict)"("Strings []"=w251) -> ()  [unwired: 2 in, 2 out]
              n167 = property on="Graph 9" class="GraphXY (strict)"("XScale.Minimum"=w249, "XScale.Maximum"=w248, "YScale.Minimum"=w247, "YScale.Maximum"=w246) -> ()  [unwired: 2 in, 2 out]
              "Régulateurs 9" <- w251
              "Graph 9" <- w252
              "Listing - 9" <- w250
            }
            frame 9 {
              # "Courbes affichées"
              n168 = for {
                tunnel: w266 -> [w267] mode=indexing
                i -> [w268]
                n169 = Increment(x=w268) -> (x+1=w269:i32)
                n170 = stacked-sequence {
                  tunnel: w267 -> [_ w271]
                  tunnel: w269 -> [w270 _]
                  frame #0 {
                    n171 = property on="Graph 10" class="GraphXY (strict)"("Active Plot"=w270) -> ()  [unwired: 2 in, 2 out]
                  }
                  frame #1 {
                    n172 = property on="Graph 10" class="GraphXY (strict)"("Plot.Visible?"=w271) -> ()  [unwired: 2 in, 2 out]
                  }
                }
              }
              n173 = property on="Tinit reg 10" class="MDér (strict)"("Strings []"=w264) -> ()  [unwired: 2 in, 2 out]
              n174 = property on="Graph 10" class="GraphXY (strict)"("XScale.Minimum"=w262, "XScale.Maximum"=w261, "YScale.Minimum"=w260, "YScale.Maximum"=w259) -> ()  [unwired: 2 in, 2 out]
              "Régulateurs 10" <- w264
              "Graph 10" <- w265
              "Listing - 10" <- w263
            }
          }
        }
        "Listings" <- w51
      }
      frame "validation" {
        w275 = TRUE ("Visible")
        n175 = property on="imprimer" class="Bool"("Visible"=w275) -> ()  [unwired: 2 in, 2 out]
        n176 = property on="Annuler" class="Bool"("Visible"=w275) -> ()  [unwired: 2 in, 2 out]
        n177 = property on="OK" class="Bool"("Visible"=w275) -> ()  [unwired: 2 in, 2 out]
        n178 = property on="Annuler lecture reg" class="Bool (strict)"("Visible"=FALSE) -> ()  [unwired: 2 in, 2 out]
        n179 = property on="Chaîne" class="Ch"("Text.BGColor"=u32 16773024 ("Texte.Couleurs du texte:Arrière-plan"), "Blinking"=FALSE ("Clignotant")) -> ()  [unwired: 2 in, 2 out]
        n180 = local write "Chaîne"("VALIDATION RUN PROFIL(S)" ("Chaîne")) -> ()
        n181 = local read "nb profils"() -> (w278:i32)
        n182 = Decrement(x=w278) -> (x-1=w277:i32)
        n183 = Not Equal To 0?(x=w277) -> (x != 0?=w276:bool)
        n184 = property on="Bascule" class="Bool (strict)"("Visible"=w276) -> ()  [unwired: 2 in, 2 out]
        n185 = while {
          tunnel: [w289] -> w282
          tunnel: w277 -> [w287]
          tunnel: w276 -> [w288]
          stop <- w290 stop-if-true
          n186 = event shown="[11] \"imprimer\": Valeur changée" {
            selector: _ -> [_ _ _ _ _ _ _ _ _ _ _ _ _ _]
            dyn-events: _ -> [_ _ _ _ _ _ _ _ _ _ _ _ _ _]
            timeout: u32 800 ("attente (ms)") -> [_ _ _ _ _ _ _ _ _ _ _ _ _ _]
            tunnel: [_ _ _ _ _ _ _ _ _ _ _ _ w549 w550] -> w290
            tunnel: [_ _ _ _ _ _ _ _ _ _ _ _ w549 _] -> w289
            tunnel: w288 -> [w295 _ _ _ _ _ _ _ _ _ _ _ _ _]
            tunnel: w287 -> [w294 _ _ _ _ _ _ _ _ _ _ _ _ _]
            event Timeout {
              n187 = event-data() -> ()  [unwired: 1 in, 3 out]
              n188 = feedback #1(u32 0 ("cas faux")) -> (w292:u32)
              n189 = And(x=w295, y="Bascule") -> (x .and. y?=w297:bool)
              n190 = case shown="Vrai" w297 {
                tunnel: w292 -> [w298 w302]
                tunnel: [w298 w300] -> w293
                tunnel: w294 -> [_ w299]
                frame False {
                }
                frame True {
                  n191 = Not Equal?(x=w302, y=w299) -> (x != y?=w304:bool)
                  n192 = Increment(x=w302) -> (x+1=w301:u32)
                  n193 = Select(t=w301, s=w304, f=u32 0 ("cas faux")) -> (s? t:f=w300:u32)
                  n194 = local write "Commande onglets"(w300) -> ()
                }
              }
              n195 = feedback-in #1(w293) -> ()
            }
            event "Tinit reg 1": Value Change {
              n196 = event-data() -> ()  [unwired: 1 in, 4 out]
              n197 = local read "Profils"() -> (w325:T2)
              n198 = Index Array(array=w325, index=0 ("indice")) -> (element=w327:T26)
              n199 = Unbundle(w327) -> ("Config + Programmes"=w328:T19, "Régulateur"=w307:T21)
              n200 = Index Array(array=w307, index="Tinit reg 1") -> (element=w322:T22)
              n201 = Unbundle By Name(w322) -> ("COM"=w323:refnum<visa-resource-name>, "Adresse"=w324:u8)
              n202 = Bundle By Name(cluster=T4 {"fractional second"=0.0, "second"=0, "minute"=0, "hour"=0, "day of month"=0, "month"=0, "year"=0, "day of week"=0, "day of year"=0, "DST"=0} ("cluster date/heure"), "hour"=1) -> (w316:T4)
              n203 = Get Date/Time In Seconds() -> (seconds since 1Jan1904=w308:timestamp)
              n204 = Date/Time To Seconds(2:w316) -> (0:w313:timestamp)  [unwired: 1 in]
              n205 = call "Acquerir valeur courante MODBUS.vi"("Adresse régulateur"=w324, "Port COM run 1 REG"=w323) -> ("Température"=w320:dbl)  [unwired: 1 out]
              n206 = Subtract(x=w308, y=w313) -> (x-y=w315:dbl)
              n207 = Build Array(w315) -> (w318:dbl[])
              n208 = Build Array(w320) -> (w319:dbl[])
              n209 = call "Generer_profil EPC3000.vi"("Temps (s)"=w318, "Num_Prog"=u8 1, "Températures (°C)"=w319, "Programmes et config"=w328) -> ("Temps (s)"=w311:dbl[], "Températures (°C)"=w310:dbl[], "Evennements_sortie"=w309:T23)  [unwired: 1 in]
              n210 = Unbundle(w328) -> ("Programmation configuration"=w321:cluster{"Command (PV)":string, dbl}[])  [unwired: 10 out]
              n211 = call "Afficher_profil.vi"("Configuration"=w321, "Temps (s)"=w311, "Températures (°C)"=w310, "Evennements_entrée"=w309) -> ("Graphe XY"=w306:cluster{"Y":dbl[], "Y":dbl[]}[])  [unwired: 3 out]
              n212 = local write "Graph 1"(w306) -> ()
            }
            event "Tinit reg 2": Value Change {
              n213 = event-data() -> ()  [unwired: 1 in, 4 out]
              n214 = local read "Profils"() -> (w349:T2)
              n215 = Index Array(array=w349, index=1 ("indice")) -> (element=w351:T26)
              n216 = Unbundle(w351) -> ("Config + Programmes"=w352:T19, "Régulateur"=w331:T21)
              n217 = Index Array(array=w331, index="Tinit reg 2") -> (element=w346:T22)
              n218 = Unbundle By Name(w346) -> ("COM"=w347:refnum<visa-resource-name>, "Adresse"=w348:u8)
              n219 = Bundle By Name(cluster=T4 {"fractional second"=0.0, "second"=0, "minute"=0, "hour"=0, "day of month"=0, "month"=0, "year"=0, "day of week"=0, "day of year"=0, "DST"=0} ("cluster date/heure"), "hour"=1) -> (w340:T4)
              n220 = Get Date/Time In Seconds() -> (seconds since 1Jan1904=w332:timestamp)
              n221 = Date/Time To Seconds(2:w340) -> (0:w337:timestamp)  [unwired: 1 in]
              n222 = call "Acquerir valeur courante MODBUS.vi"("Adresse régulateur"=w348, "Port COM run 1 REG"=w347) -> ("Température"=w344:dbl)  [unwired: 1 out]
              n223 = Subtract(x=w332, y=w337) -> (x-y=w339:dbl)
              n224 = Build Array(w339) -> (w342:dbl[])
              n225 = Build Array(w344) -> (w343:dbl[])
              n226 = call "Generer_profil EPC3000.vi"("Temps (s)"=w342, "Num_Prog"=u8 1, "Températures (°C)"=w343, "Programmes et config"=w352) -> ("Temps (s)"=w335:dbl[], "Températures (°C)"=w334:dbl[], "Evennements_sortie"=w333:T23)  [unwired: 1 in]
              n227 = Unbundle(w352) -> ("Programmation configuration"=w345:cluster{"Command (PV)":string, dbl}[])  [unwired: 10 out]
              n228 = call "Afficher_profil.vi"("Configuration"=w345, "Temps (s)"=w335, "Températures (°C)"=w334, "Evennements_entrée"=w333) -> ("Graphe XY"=w330:cluster{"Y":dbl[], "Y":dbl[]}[])  [unwired: 3 out]
              n229 = local write "Graph 2"(w330) -> ()
            }
            event "Tinit reg 3": Value Change {
              n230 = event-data() -> ()  [unwired: 1 in, 4 out]
              n231 = local read "Profils"() -> (w373:T2)
              n232 = Index Array(array=w373, index=2 ("indice")) -> (element=w375:T26)
              n233 = Unbundle(w375) -> ("Config + Programmes"=w376:T19, "Régulateur"=w355:T21)
              n234 = Index Array(array=w355, index="Tinit reg 3") -> (element=w370:T22)
              n235 = Unbundle By Name(w370) -> ("COM"=w371:refnum<visa-resource-name>, "Adresse"=w372:u8)
              n236 = Bundle By Name(cluster=T4 {"fractional second"=0.0, "second"=0, "minute"=0, "hour"=0, "day of month"=0, "month"=0, "year"=0, "day of week"=0, "day of year"=0, "DST"=0} ("cluster date/heure"), "hour"=1) -> (w364:T4)
              n237 = Get Date/Time In Seconds() -> (seconds since 1Jan1904=w356:timestamp)
              n238 = Date/Time To Seconds(2:w364) -> (0:w361:timestamp)  [unwired: 1 in]
              n239 = call "Acquerir valeur courante MODBUS.vi"("Adresse régulateur"=w372, "Port COM run 1 REG"=w371) -> ("Température"=w368:dbl)  [unwired: 1 out]
              n240 = Subtract(x=w356, y=w361) -> (x-y=w363:dbl)
              n241 = Build Array(w363) -> (w366:dbl[])
              n242 = Build Array(w368) -> (w367:dbl[])
              n243 = call "Generer_profil EPC3000.vi"("Temps (s)"=w366, "Num_Prog"=u8 1, "Températures (°C)"=w367, "Programmes et config"=w376) -> ("Temps (s)"=w359:dbl[], "Températures (°C)"=w358:dbl[], "Evennements_sortie"=w357:T23)  [unwired: 1 in]
              n244 = Unbundle(w376) -> ("Programmation configuration"=w369:cluster{"Command (PV)":string, dbl}[])  [unwired: 10 out]
              n245 = call "Afficher_profil.vi"("Configuration"=w369, "Temps (s)"=w359, "Températures (°C)"=w358, "Evennements_entrée"=w357) -> ("Graphe XY"=w354:cluster{"Y":dbl[], "Y":dbl[]}[])  [unwired: 3 out]
              n246 = local write "Graph 3"(w354) -> ()
            }
            event "Tinit reg 4": Value Change {
              n247 = event-data() -> ()  [unwired: 1 in, 4 out]
              n248 = local read "Profils"() -> (w397:T2)
              n249 = Index Array(array=w397, index=3 ("indice")) -> (element=w399:T26)
              n250 = Unbundle(w399) -> ("Config + Programmes"=w400:T19, "Régulateur"=w379:T21)
              n251 = Index Array(array=w379, index="Tinit reg 4") -> (element=w394:T22)
              n252 = Unbundle By Name(w394) -> ("COM"=w395:refnum<visa-resource-name>, "Adresse"=w396:u8)
              n253 = Bundle By Name(cluster=T4 {"fractional second"=0.0, "second"=0, "minute"=0, "hour"=0, "day of month"=0, "month"=0, "year"=0, "day of week"=0, "day of year"=0, "DST"=0} ("cluster date/heure"), "hour"=1) -> (w388:T4)
              n254 = Get Date/Time In Seconds() -> (seconds since 1Jan1904=w380:timestamp)
              n255 = Date/Time To Seconds(2:w388) -> (0:w385:timestamp)  [unwired: 1 in]
              n256 = call "Acquerir valeur courante MODBUS.vi"("Adresse régulateur"=w396, "Port COM run 1 REG"=w395) -> ("Température"=w392:dbl)  [unwired: 1 out]
              n257 = Subtract(x=w380, y=w385) -> (x-y=w387:dbl)
              n258 = Build Array(w387) -> (w390:dbl[])
              n259 = Build Array(w392) -> (w391:dbl[])
              n260 = call "Generer_profil EPC3000.vi"("Temps (s)"=w390, "Num_Prog"=u8 1, "Températures (°C)"=w391, "Programmes et config"=w400) -> ("Temps (s)"=w383:dbl[], "Températures (°C)"=w382:dbl[], "Evennements_sortie"=w381:T23)  [unwired: 1 in]
              n261 = Unbundle(w400) -> ("Programmation configuration"=w393:cluster{"Command (PV)":string, dbl}[])  [unwired: 10 out]
              n262 = call "Afficher_profil.vi"("Configuration"=w393, "Temps (s)"=w383, "Températures (°C)"=w382, "Evennements_entrée"=w381) -> ("Graphe XY"=w378:cluster{"Y":dbl[], "Y":dbl[]}[])  [unwired: 3 out]
              n263 = local write "Graph 4"(w378) -> ()
            }
            event "Tinit reg 5": Value Change {
              n264 = event-data() -> ()  [unwired: 1 in, 4 out]
              n265 = local read "Profils"() -> (w421:T2)
              n266 = Index Array(array=w421, index=4 ("indice")) -> (element=w423:T26)
              n267 = Unbundle(w423) -> ("Config + Programmes"=w424:T19, "Régulateur"=w403:T21)
              n268 = Index Array(array=w403, index="Tinit reg 5") -> (element=w418:T22)
              n269 = Unbundle By Name(w418) -> ("COM"=w419:refnum<visa-resource-name>, "Adresse"=w420:u8)
              n270 = Bundle By Name(cluster=T4 {"fractional second"=0.0, "second"=0, "minute"=0, "hour"=0, "day of month"=0, "month"=0, "year"=0, "day of week"=0, "day of year"=0, "DST"=0} ("cluster date/heure"), "hour"=1) -> (w412:T4)
              n271 = Get Date/Time In Seconds() -> (seconds since 1Jan1904=w404:timestamp)
              n272 = Date/Time To Seconds(2:w412) -> (0:w409:timestamp)  [unwired: 1 in]
              n273 = call "Acquerir valeur courante MODBUS.vi"("Adresse régulateur"=w420, "Port COM run 1 REG"=w419) -> ("Température"=w416:dbl)  [unwired: 1 out]
              n274 = Subtract(x=w404, y=w409) -> (x-y=w411:dbl)
              n275 = Build Array(w411) -> (w414:dbl[])
              n276 = Build Array(w416) -> (w415:dbl[])
              n277 = call "Generer_profil EPC3000.vi"("Temps (s)"=w414, "Num_Prog"=u8 1, "Températures (°C)"=w415, "Programmes et config"=w424) -> ("Temps (s)"=w407:dbl[], "Températures (°C)"=w406:dbl[], "Evennements_sortie"=w405:T23)  [unwired: 1 in]
              n278 = Unbundle(w424) -> ("Programmation configuration"=w417:cluster{"Command (PV)":string, dbl}[])  [unwired: 10 out]
              n279 = call "Afficher_profil.vi"("Configuration"=w417, "Temps (s)"=w407, "Températures (°C)"=w406, "Evennements_entrée"=w405) -> ("Graphe XY"=w402:cluster{"Y":dbl[], "Y":dbl[]}[])  [unwired: 3 out]
              n280 = local write "Graph 5"(w402) -> ()
            }
            event "Tinit reg 6": Value Change {
              n281 = event-data() -> ()  [unwired: 1 in, 4 out]
              n282 = local read "Profils"() -> (w445:T2)
              n283 = Index Array(array=w445, index=5 ("indice")) -> (element=w447:T26)
              n284 = Unbundle(w447) -> ("Config + Programmes"=w448:T19, "Régulateur"=w427:T21)
              n285 = Index Array(array=w427, index="Tinit reg 6") -> (element=w442:T22)
              n286 = Unbundle By Name(w442) -> ("COM"=w443:refnum<visa-resource-name>, "Adresse"=w444:u8)
              n287 = Bundle By Name(cluster=T4 {"fractional second"=0.0, "second"=0, "minute"=0, "hour"=0, "day of month"=0, "month"=0, "year"=0, "day of week"=0, "day of year"=0, "DST"=0} ("cluster date/heure"), "hour"=1) -> (w436:T4)
              n288 = Get Date/Time In Seconds() -> (seconds since 1Jan1904=w428:timestamp)
              n289 = Date/Time To Seconds(2:w436) -> (0:w433:timestamp)  [unwired: 1 in]
              n290 = call "Acquerir valeur courante MODBUS.vi"("Adresse régulateur"=w444, "Port COM run 1 REG"=w443) -> ("Température"=w440:dbl)  [unwired: 1 out]
              n291 = Subtract(x=w428, y=w433) -> (x-y=w435:dbl)
              n292 = Build Array(w435) -> (w438:dbl[])
              n293 = Build Array(w440) -> (w439:dbl[])
              n294 = call "Generer_profil EPC3000.vi"("Temps (s)"=w438, "Num_Prog"=u8 1, "Températures (°C)"=w439, "Programmes et config"=w448) -> ("Temps (s)"=w431:dbl[], "Températures (°C)"=w430:dbl[], "Evennements_sortie"=w429:T23)  [unwired: 1 in]
              n295 = Unbundle(w448) -> ("Programmation configuration"=w441:cluster{"Command (PV)":string, dbl}[])  [unwired: 10 out]
              n296 = call "Afficher_profil.vi"("Configuration"=w441, "Temps (s)"=w431, "Températures (°C)"=w430, "Evennements_entrée"=w429) -> ("Graphe XY"=w426:cluster{"Y":dbl[], "Y":dbl[]}[])  [unwired: 3 out]
              n297 = local write "Graph 6"(w426) -> ()
            }
            event "Tinit reg 7": Value Change {
              n298 = event-data() -> ()  [unwired: 1 in, 4 out]
              n299 = local read "Profils"() -> (w469:T2)
              n300 = Index Array(array=w469, index=6 ("indice")) -> (element=w471:T26)
              n301 = Unbundle(w471) -> ("Config + Programmes"=w472:T19, "Régulateur"=w451:T21)
              n302 = Index Array(array=w451, index="Tinit reg 7") -> (element=w466:T22)
              n303 = Unbundle By Name(w466) -> ("COM"=w467:refnum<visa-resource-name>, "Adresse"=w468:u8)
              n304 = Bundle By Name(cluster=T4 {"fractional second"=0.0, "second"=0, "minute"=0, "hour"=0, "day of month"=0, "month"=0, "year"=0, "day of week"=0, "day of year"=0, "DST"=0} ("cluster date/heure"), "hour"=1) -> (w460:T4)
              n305 = Get Date/Time In Seconds() -> (seconds since 1Jan1904=w452:timestamp)
              n306 = Date/Time To Seconds(2:w460) -> (0:w457:timestamp)  [unwired: 1 in]
              n307 = call "Acquerir valeur courante MODBUS.vi"("Adresse régulateur"=w468, "Port COM run 1 REG"=w467) -> ("Température"=w464:dbl)  [unwired: 1 out]
              n308 = Subtract(x=w452, y=w457) -> (x-y=w459:dbl)
              n309 = Build Array(w459) -> (w462:dbl[])
              n310 = Build Array(w464) -> (w463:dbl[])
              n311 = call "Generer_profil EPC3000.vi"("Temps (s)"=w462, "Num_Prog"=u8 1, "Températures (°C)"=w463, "Programmes et config"=w472) -> ("Temps (s)"=w455:dbl[], "Températures (°C)"=w454:dbl[], "Evennements_sortie"=w453:T23)  [unwired: 1 in]
              n312 = Unbundle(w472) -> ("Programmation configuration"=w465:cluster{"Command (PV)":string, dbl}[])  [unwired: 10 out]
              n313 = call "Afficher_profil.vi"("Configuration"=w465, "Temps (s)"=w455, "Températures (°C)"=w454, "Evennements_entrée"=w453) -> ("Graphe XY"=w450:cluster{"Y":dbl[], "Y":dbl[]}[])  [unwired: 3 out]
              n314 = local write "Graph 7"(w450) -> ()
            }
            event "Tinit reg 8": Value Change {
              n315 = event-data() -> ()  [unwired: 1 in, 4 out]
              n316 = local read "Profils"() -> (w493:T2)
              n317 = Index Array(array=w493, index=7 ("indice")) -> (element=w495:T26)
              n318 = Unbundle(w495) -> ("Config + Programmes"=w496:T19, "Régulateur"=w475:T21)
              n319 = Index Array(array=w475, index="Tinit reg 8") -> (element=w490:T22)
              n320 = Unbundle By Name(w490) -> ("COM"=w491:refnum<visa-resource-name>, "Adresse"=w492:u8)
              n321 = Bundle By Name(cluster=T4 {"fractional second"=0.0, "second"=0, "minute"=0, "hour"=0, "day of month"=0, "month"=0, "year"=0, "day of week"=0, "day of year"=0, "DST"=0} ("cluster date/heure"), "hour"=1) -> (w484:T4)
              n322 = Get Date/Time In Seconds() -> (seconds since 1Jan1904=w476:timestamp)
              n323 = Date/Time To Seconds(2:w484) -> (0:w481:timestamp)  [unwired: 1 in]
              n324 = call "Acquerir valeur courante MODBUS.vi"("Adresse régulateur"=w492, "Port COM run 1 REG"=w491) -> ("Température"=w488:dbl)  [unwired: 1 out]
              n325 = Subtract(x=w476, y=w481) -> (x-y=w483:dbl)
              n326 = Build Array(w483) -> (w486:dbl[])
              n327 = Build Array(w488) -> (w487:dbl[])
              n328 = call "Generer_profil EPC3000.vi"("Temps (s)"=w486, "Num_Prog"=u8 1, "Températures (°C)"=w487, "Programmes et config"=w496) -> ("Temps (s)"=w479:dbl[], "Températures (°C)"=w478:dbl[], "Evennements_sortie"=w477:T23)  [unwired: 1 in]
              n329 = Unbundle(w496) -> ("Programmation configuration"=w489:cluster{"Command (PV)":string, dbl}[])  [unwired: 10 out]
              n330 = call "Afficher_profil.vi"("Configuration"=w489, "Temps (s)"=w479, "Températures (°C)"=w478, "Evennements_entrée"=w477) -> ("Graphe XY"=w474:cluster{"Y":dbl[], "Y":dbl[]}[])  [unwired: 3 out]
              n331 = local write "Graph 8"(w474) -> ()
            }
            event "Tinit reg 9": Value Change {
              n332 = event-data() -> ()  [unwired: 1 in, 4 out]
              n333 = local read "Profils"() -> (w517:T2)
              n334 = Index Array(array=w517, index=8 ("indice")) -> (element=w519:T26)
              n335 = Unbundle(w519) -> ("Config + Programmes"=w520:T19, "Régulateur"=w499:T21)
              n336 = Index Array(array=w499, index="Tinit reg 9") -> (element=w514:T22)
              n337 = Unbundle By Name(w514) -> ("COM"=w515:refnum<visa-resource-name>, "Adresse"=w516:u8)
              n338 = Bundle By Name(cluster=T4 {"fractional second"=0.0, "second"=0, "minute"=0, "hour"=0, "day of month"=0, "month"=0, "year"=0, "day of week"=0, "day of year"=0, "DST"=0} ("cluster date/heure"), "hour"=1) -> (w508:T4)
              n339 = Get Date/Time In Seconds() -> (seconds since 1Jan1904=w500:timestamp)
              n340 = Date/Time To Seconds(2:w508) -> (0:w505:timestamp)  [unwired: 1 in]
              n341 = call "Acquerir valeur courante MODBUS.vi"("Adresse régulateur"=w516, "Port COM run 1 REG"=w515) -> ("Température"=w512:dbl)  [unwired: 1 out]
              n342 = Subtract(x=w500, y=w505) -> (x-y=w507:dbl)
              n343 = Build Array(w507) -> (w510:dbl[])
              n344 = Build Array(w512) -> (w511:dbl[])
              n345 = call "Generer_profil EPC3000.vi"("Temps (s)"=w510, "Num_Prog"=u8 1, "Températures (°C)"=w511, "Programmes et config"=w520) -> ("Temps (s)"=w503:dbl[], "Températures (°C)"=w502:dbl[], "Evennements_sortie"=w501:T23)  [unwired: 1 in]
              n346 = Unbundle(w520) -> ("Programmation configuration"=w513:cluster{"Command (PV)":string, dbl}[])  [unwired: 10 out]
              n347 = call "Afficher_profil.vi"("Configuration"=w513, "Temps (s)"=w503, "Températures (°C)"=w502, "Evennements_entrée"=w501) -> ("Graphe XY"=w498:cluster{"Y":dbl[], "Y":dbl[]}[])  [unwired: 3 out]
              n348 = local write "Graph 9"(w498) -> ()
            }
            event "Tinit reg 10": Value Change {
              n349 = event-data() -> ()  [unwired: 1 in, 4 out]
              n350 = local read "Profils"() -> (w541:T2)
              n351 = Index Array(array=w541, index=9 ("indice")) -> (element=w543:T26)
              n352 = Unbundle(w543) -> ("Config + Programmes"=w544:T19, "Régulateur"=w523:T21)
              n353 = Index Array(array=w523, index="Tinit reg 10") -> (element=w538:T22)
              n354 = Unbundle By Name(w538) -> ("COM"=w539:refnum<visa-resource-name>, "Adresse"=w540:u8)
              n355 = Bundle By Name(cluster=T4 {"fractional second"=0.0, "second"=0, "minute"=0, "hour"=0, "day of month"=0, "month"=0, "year"=0, "day of week"=0, "day of year"=0, "DST"=0} ("cluster date/heure"), "hour"=1) -> (w532:T4)
              n356 = Get Date/Time In Seconds() -> (seconds since 1Jan1904=w524:timestamp)
              n357 = Date/Time To Seconds(2:w532) -> (0:w529:timestamp)  [unwired: 1 in]
              n358 = call "Acquerir valeur courante MODBUS.vi"("Adresse régulateur"=w540, "Port COM run 1 REG"=w539) -> ("Température"=w536:dbl)  [unwired: 1 out]
              n359 = Subtract(x=w524, y=w529) -> (x-y=w531:dbl)
              n360 = Build Array(w531) -> (w534:dbl[])
              n361 = Build Array(w536) -> (w535:dbl[])
              n362 = call "Generer_profil EPC3000.vi"("Temps (s)"=w534, "Num_Prog"=u8 1, "Températures (°C)"=w535, "Programmes et config"=w544) -> ("Temps (s)"=w527:dbl[], "Températures (°C)"=w526:dbl[], "Evennements_sortie"=w525:T23)  [unwired: 1 in]
              n363 = Unbundle(w544) -> ("Programmation configuration"=w537:cluster{"Command (PV)":string, dbl}[])  [unwired: 10 out]
              n364 = call "Afficher_profil.vi"("Configuration"=w537, "Temps (s)"=w527, "Températures (°C)"=w526, "Evennements_entrée"=w525) -> ("Graphe XY"=w522:cluster{"Y":dbl[], "Y":dbl[]}[])  [unwired: 3 out]
              n365 = local write "Graph 10"(w522) -> ()
            }
            event "imprimer": Value Change {
              w545 = T27 0 items=["Impression rapide", "Rapport standard", "HTML", "Word", "Excel"] ("report type (Quick Print)")
              w546 = T28 1 items=["Face-avant complète", "Partie visible de la face-avant", "Icône, description, face-avant et diagramme", "Doumentation : Orientée face-avant", "Documentation : Orientée sous-VI", "Documentation : Complète", "Documentation : personnalisée"] ("contents (complete front panel)")
              n366 = event-data() -> ()  [unwired: 1 in, 3 out]
              n367 = call "Chemin VI actuel (VI or exe).vi"() -> ("Full Path to VI or executable"=w547:path)  [unwired: 14 in, 1 out]
              n368 = call-poly <vilib>:"Print VI Panel or Documentation.vi"("layout options"=T5 {"orientation (unchanged)"=1, "panel scaling for page (unchanged)"=2, "margins"={"override VI margins (false)"=FALSE, "margins (1.00)"={"top"=1.0, "left"=1.0, "right"=1.0, "bottom"=1.0}, "measurement system (default)"=2}, "printer options"={"destination printer name (current)"="", "printing method (unchanged)"=1, "color or monochrome (unchanged)"=1}, "page header options"={"page headers (unchanged)"=2, "page header content options"={"Include VI Name"=FALSE, "Include VI Path"=FALSE, "Include Last Modification Date"=FALSE, "Include Date Printed"=FALSE, "Include Page Number"=FALSE, "Include VI Icon"=FALSE}}}, "report type (Quick Print)"=w545, "contents (complete front panel)"=w546, "VI path"=w547) -> ()  [unwired: 6 in, 2 out]
            }
            event "OK": Value Change {
              n369 = event-data() -> ("NewVal"=w549:bool)  [unwired: 1 in, 5 out]
            }
            event "Annuler": Value Change {
              n370 = event-data() -> ("NewVal"=w550:bool)  [unwired: 1 in, 5 out]
              "annulé" <- w550
            }
          }
        }
        n371 = Select(t=Enum_r3."fichiers images graph" ("Énum"), s=w282, f=Enum_r3."fin" ("Énum")) -> (s? t:f=w283:T3)
      }
      frame "fichiers images graph" {
        n372 = Strip Path(path="Chemin du fichier rapport") -> (stripped path=w558:path, name=w559:string)
        n373 = call <vilib>:"Check if File or Folder Exists.vi"("path"=w558) -> ("file or folder exists?"=w557:bool)  [unwired: 8 in, 2 out]
        n374 = property on="Chaîne" class="Ch"("Text.BGColor"=u32 16728642 ("Texte.Couleurs du texte:Arrière-plan"), "Blinking"=TRUE ("Clignotant")) -> ()  [unwired: 2 in, 2 out]
        n375 = case shown="Vrai" w557 {
          tunnel: w558 -> [w598 _]
          tunnel: [w595 w599] -> w556
          tunnel: w559 -> [w596 _]
          tunnel: "Chemin du fichier rapport" -> [_ w599]
          frame False {
            n376 = Create Folder(path (use dialog)=w598) -> (created path=w597:path)  [unwired: 2 in, 2 out]
            n377 = Build Path(base path=w597, name or relative path=w596) -> (appended path=w595:path)
          }
          frame True {
          }
        }
        n378 = local write "Chaîne"("CRÉATION DU FICHIER HTML" ("Chaîne")) -> ()
        n379 = local read "nb profils"() -> (w551:i32)
        n380 = for {
          N: w551 -> [_]
          tunnel: w556 -> [w564]
          tunnel: [w563] -> w555 mode=indexing
          i -> [w562]
          # "Sauvegarde de l'image du profil"
          n381 = Path To String(path=w564) -> (string=w573:string)
          n382 = String Length(string=w573) -> (length=w572:i32)
          n383 = Increment(x=w562) -> (x+1=w569:i32)
          n384 = Subtract(x=w572, y=4) -> (x-y=w570:i32)
          n385 = Number To Decimal String(number=w569) -> (decimal integer string=w567:string)  [unwired: 1 in]
          n386 = String Subset(string=w573, length (rest)=w570) -> (substring=w574:string)  [unwired: 1 in]
          n387 = Concatenate Strings(w574, "_Profil_n°" ("chaîne"), w567, ".bmp" ("chaîne")) -> (w565:string)
          n388 = String To Path(string=w565) -> (path=w563:path)
          n389 = case shown="0, Par défaut" w562 {
            tunnel: w563 -> [w575 w579 w583 w587 w591]
            frame 0, Default {
              w576 = FALSE ("Masquer la grille")
              n390 = invoke on="Graph 1" class="GraphXY (strict)" method="ExportImage"("FileType"=enum32{"BMP", "EPS", "EMF", "PICT"}."BMP" ("Type de fichier"), "Target"=enum32{"File", "Clipboard"}."File" ("Destination"), "Path"=w575, "HideGrid"=w576, "Overwrite"=w576) -> ()  [unwired: 3 in, 8 out]
            }
            frame 1 {
              w580 = FALSE ("Masquer la grille")
              n391 = invoke on="Graph 2" class="GraphXY (strict)" method="ExportImage"("FileType"=enum32{"BMP", "EPS", "EMF", "PICT"}."BMP" ("Type de fichier"), "Target"=enum32{"File", "Clipboard"}."File" ("Destination"), "Path"=w579, "HideGrid"=w580, "Overwrite"=w580) -> ()  [unwired: 3 in, 8 out]
            }
            frame 2 {
              w584 = FALSE ("Masquer la grille")
              n392 = invoke on="Graph 3" class="GraphXY (strict)" method="ExportImage"("FileType"=enum32{"BMP", "EPS", "EMF", "PICT"}."BMP" ("Type de fichier"), "Target"=enum32{"File", "Clipboard"}."File" ("Destination"), "Path"=w583, "HideGrid"=w584, "Overwrite"=w584) -> ()  [unwired: 3 in, 8 out]
            }
            frame 3 {
              w588 = FALSE ("Masquer la grille")
              n393 = invoke on="Graph 4" class="GraphXY (strict)" method="ExportImage"("FileType"=enum32{"BMP", "EPS", "EMF", "PICT"}."BMP" ("Type de fichier"), "Target"=enum32{"File", "Clipboard"}."File" ("Destination"), "Path"=w587, "HideGrid"=w588, "Overwrite"=w588) -> ()  [unwired: 3 in, 8 out]
            }
            frame 4 {
              w592 = FALSE ("Masquer la grille")
              n394 = invoke on="Graph 5" class="GraphXY (strict)" method="ExportImage"("FileType"=enum32{"BMP", "EPS", "EMF", "PICT"}."BMP" ("Type de fichier"), "Target"=enum32{"File", "Clipboard"}."File" ("Destination"), "Path"=w591, "HideGrid"=w592, "Overwrite"=w592) -> ()  [unwired: 3 in, 8 out]
            }
          }
        }
        "fichiers images" <- w555
      }
      frame "fichier html" {
        n395 = Get Date/Time In Seconds() -> (seconds since 1Jan1904=w622:timestamp)
        n396 = Get Date/Time String(date format (0)=enum16{"short", "long", "abbreviated"}."long" ("format de date (0)"), seconds (now)=w622, want seconds? (F)=TRUE ("secondes ? (F)")) -> (date string=w606:string, time string=w605:string)
        n397 = Format Into String(format string="<h1><center>- Fichier Profil -</center></h1></br><hr><h2>Commentaires :</h2>%s</br><hr><h2>Mise en RUN : </h2></br>%s</br>%s</br><hr>" ("chaîne de format"), "Commentaires", w606, w605) -> (resulting string=w604:string)  [unwired: 2 in, 1 out]
        n398 = call <vilib>:"New Report.vi"("report type"=T17."HTML") -> ("report out"=w620:refnum<class "NI_report.lvclass">, "error out"=w621:errorcluster)  [unwired: 13 in]
        n399 = local read "Profils"() -> (w614:T2)
        n400 = call-dynamic "Append User Formatted HTML to Report.vi"("report in"=w620, "HTML text"=w604, "error in (no error)"=w621) -> ("report out"=w603:refnum<class "NI_report.lvclass">, "error out"=w602:errorcluster)  [unwired: 11 in]
        n401 = local read "Listings"() -> (w615:string[])
        n402 = local read "fichiers images"() -> (w613:path[])
        n403 = for {
          tunnel: w615 -> [w636] mode=indexing
          tunnel: w614 -> [w635] mode=indexing
          tunnel: w613 -> [w633] mode=indexing
          shift-right: [w629] -> w608
          shift-left: w602 -> [w628]
          shift-right: [w630] -> w609
          shift-left: w603 -> [w627]
          i -> [w637]
          w651 = "\r\n"
          # "sauvegarde fichier html"
          # "Listing"
          # "chemin img"
          n404 = Unbundle(w635) -> ("Régulateur"=w634:T21)  [unwired: 1 out]
          n405 = for {
            tunnel: w634 -> [w653] mode=indexing
            shift-right: [w655] -> w624
            shift-left: "" -> [w656]
            n406 = Unbundle(w653) -> ("Nom"=w652:string)  [unwired: 2 out]
            n407 = Concatenate Strings(w656, "</br>", w652) -> (w655:string)
          }
          n408 = Increment(x=w637) -> (x+1=w625:i32)
          n409 = Format Into String(format string="<h2>Profil de r\\E9gulation n\\B0%d</h2></br><h3>Appliqu\\E9 au(x) r\\E9gulateur(s) suivant(s) : %s</h3></br>" ("chaîne de format"), w625, w624) -> (resulting string=w623:string)  [unwired: 2 in, 1 out]
          n410 = call-dynamic "Append User Formatted HTML to Report.vi"("report in"=w627, "HTML text"=w623, "error in (no error)"=w628) -> ("report out"=w642:refnum<class "NI_report.lvclass">, "error out"=w641:errorcluster)  [unwired: 11 in]
          n411 = call-poly <vilib>:"Append Report Text.vi"("report in"=w642, "text"=w636, "append on new line? (F)"=TRUE, "error in (no error)"=w641) -> ("report out"=w644:refnum<class "NI_report.lvclass">, "error out"=w647:errorcluster)  [unwired: 8 in, 2 out]
          n412 = Concatenate Strings(w651, "Profil : " ("text"), w651) -> (w649:string)
          n413 = call-poly <vilib>:"Append Report Text.vi"("report in"=w644, "text"=w649, "append on new line? (F)"=TRUE, "error in (no error)"=w647) -> ("report out"=w645:refnum<class "NI_report.lvclass">, "error out"=w646:errorcluster)  [unwired: 8 in, 2 out]
          n414 = call-poly <vilib>:"Append Image to Report.vi"("report in"=w645, "alignment (default)"=HTML_Report_Image_Alignment."MIDDLE", "path or URL of image"=w633, "caption or alternative string"="Profil de régulation", "error in (no error)"=w646) -> ("report out"=w632:refnum<class "NI_report.lvclass">, "error out"=w631:errorcluster)  [unwired: 7 in, 2 out]
          n415 = call-dynamic "Append Horizontal Line to Report.vi"("report in"=w632, "error in (no error)"=w631) -> ("report out"=w630:refnum<class "NI_report.lvclass">, "error out"=w629:errorcluster)  [unwired: 12 in]
        }
        n416 = local read "Chemin du fichier rapport"() -> (w601:path)
        n417 = call-dynamic "Save Report to File.vi"("report in"=w609, "report file path"=w601, "error in (no error)"=w608) -> ("report out"=w611:refnum<class "NI_report.lvclass">, "error out"=w610:errorcluster)  [unwired: 11 in]
        n418 = call-dynamic "Dispose Report.vi"("report in"=w611, "error in (no error)"=w610) -> ("error out"=→"error out":errorcluster)  [unwired: 13 in]
      }
      frame "fin" {
        n419 = Request Deallocation(TRUE ("flag")) -> ()
      }
    }
  }
